vi "GpuMat AdjustRoi.vi"(8 "error in (no error)":errorcluster, 10 "Delta":T1, 11 "Src in":refnum<class "GpuMat.lvclass">) -> (0 "error out":errorcluster, 3 "Src out":refnum<class "GpuMat.lvclass">)   [LabVIEW 2020, in "OpenLvVision_OpenCv.lvlib" / "Cuda.lvlib" / "GpuMat.lvclass"]
doc: "moves/resizes the current GpuMat ROI inside the parent GpuMat"
uses:
  GpuMat.lvclass
  <vilib>/Utility/error.llb/Error Cluster From Error Code.vi
  <vilib>/ErrorRing/Error Ring.xnode
  OpenLvVision_OpenCv.lvlib
  _LvHelpers/EdvrObject/EdvrObject.lvclass
  Dlls/OlvOpenCvWrapper.dll
  C:/Users/lukas/Documents/OpenLvVision_OpenCv/SourceCode/LabView/OpenLvVision_OpenCv/_LvHelpers/EdvrObject/EdvrObject.lvclass
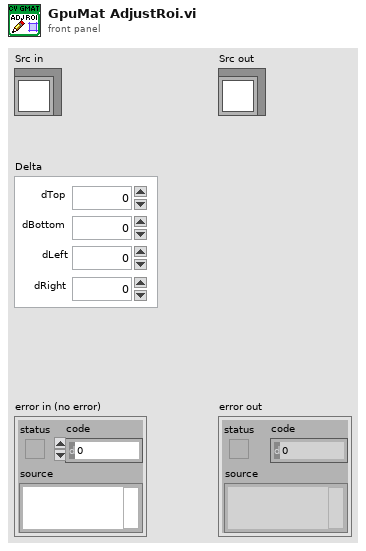
[diagram p1: front panel]
types:
  T1 = cluster{"dTop":i32, "dBottom":i32, "dLeft":i32, "dRight":i32}
  T2 = typedef "OpenLvVision_OpenCv.lvlib/EdvrObject.lvclass/Edvr.ctl" = refnum<data-value>
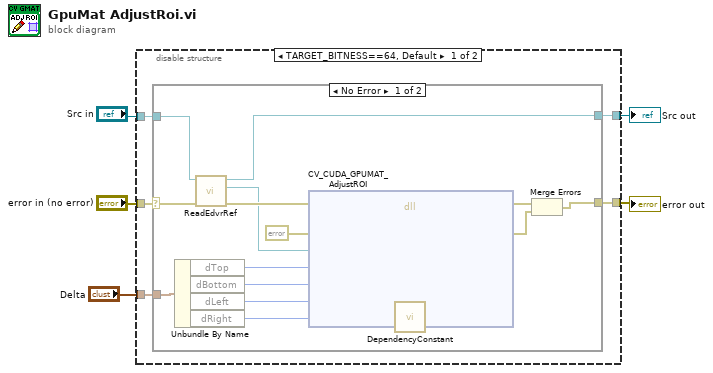
[diagram p0: block diagram]
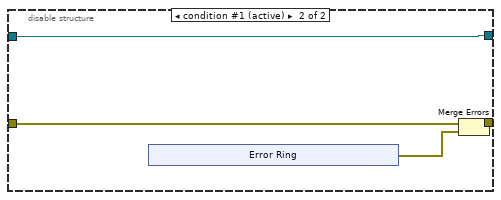
[diagram p3: hidden frame]
diagram:
  n1 = disable-structure shown="TARGET_BITNESS==64, Default" {
    disable-tunnel: "error in (no error)" -> [w10 w29]
    disable-tunnel: [w9 w30] -> w5
    disable-tunnel: "Src in" -> [w8 w27]
    disable-tunnel: [w7 w27] -> w2
    disable-tunnel: "Delta" -> [w6 _]
    frame condition #0 {
      n2 = case shown="No Error" w10 {
        selector: w10 -> [w17 w26]
        tunnel: [w16 w26] -> w9
        tunnel: w8 -> [w19 w25]
        tunnel: [w18 w25] -> w7
        tunnel: w6 -> [w15 _]
        frame No Error {
          n3 = Unbundle By Name(w15) -> ("dTop"=w14:i32, "dBottom"=w13:i32, "dLeft"=w12:i32, "dRight"=w11:i32)
          n4 = call "ReadEdvrRef.vi"("error in (no error)"=w17, "EdvrObject in"=w19) -> ("error out"=w21:errorcluster, "Edvr"=w20:T2, "EdvrObject out"=w18:refnum<class "GpuMat.lvclass">)  [unwired: 7 in]
          n5 = dll-call lib="C:/Users/lukas/Documents/OpenLvVision_OpenCv/SourceCode/LabView/OpenLvVision_OpenCv/Dlls/OlvOpenCvWrapper.dll" fn="CV_CUDA_GPUMAT_AdjustROI"(error in=w21, "Error"=errorcluster {"status"=FALSE, "code"=0, "source"=""} ("error out"), "srcRef"=w20, "dtop"=w14, "dbottom"=w13, "dleft"=w12, "dright"=w11) -> (error out=w24:errorcluster, "Error"=w23:errorcluster)  [unwired: 8 in, 1 out]
          n6 = call "DependencyConstant.vi"() -> ()  [unwired: 12 in]
          n7 = Merge Errors(w24, w23) -> (w16:errorcluster)
        }
        frame Error {
        }
      }
    }
    frame condition #1 (active) {
      n8 = xnode "Error Ring"() -> ("error out"=w28:errorcluster)
      n9 = Merge Errors(w29, w28) -> (w30:errorcluster)
    }
  }
  "error out" <- w5
  "Src out" <- w2
